vi "get_edge_attribute.vi"(7 "attribute-name":string, 8 "error in (no error)":errorcluster, 9 "default value (empty variant)":variant, 10 "edge":refnum<class "Edge.lvclass">, 11 "graph":refnum<class "Graph.lvclass">) -> (0 "error out":errorcluster, 1 "attribute-value":variant, 2 "attribute-found":bool, 3 "graph-out":refnum<class "Graph.lvclass">)   [LabVIEW 2020, in "graph.lvlib" / "Graph.lvclass"]
uses:
  Graph.lvclass
  Edge/Edge.lvclass
  Graph.lvclass/Graph.ctl
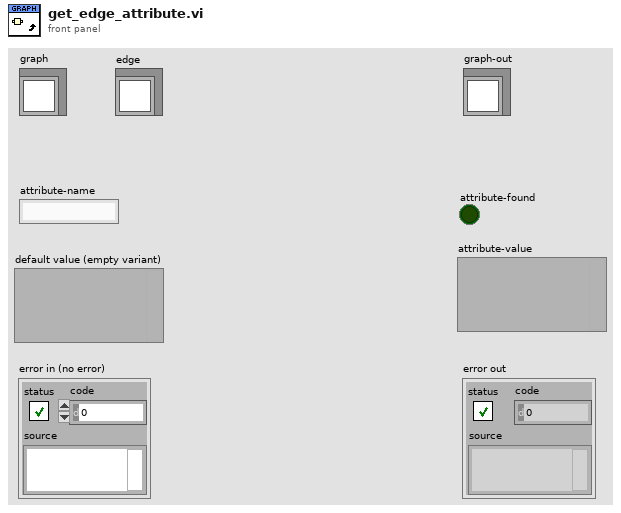
[diagram p1: front panel]
types:
  T1 = typedef "graph.lvlib/Graph.lvclass/edge-definition-cluster.ctl" = cluster{"source-id":refnum<class "ID.lvclass">, "sink-id":refnum<class "ID.lvclass">}
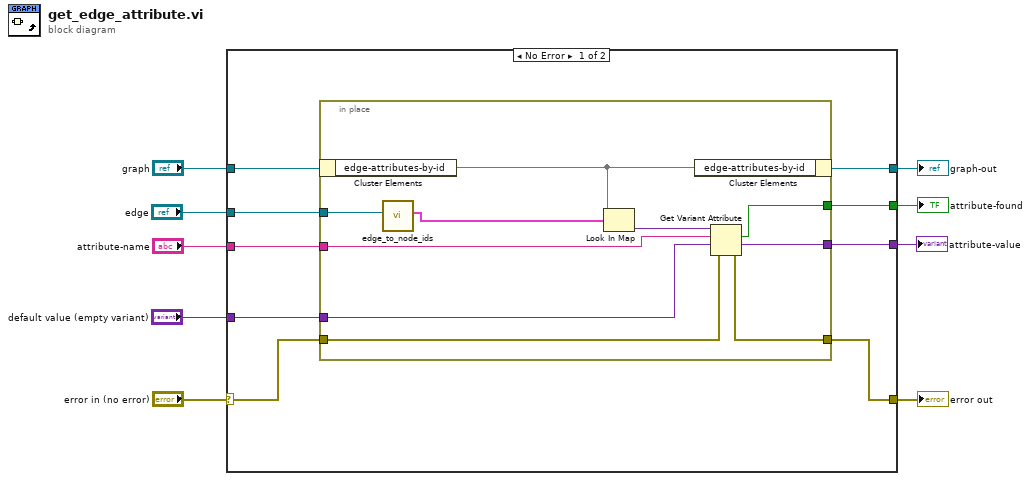
[diagram p0: block diagram]
diagram:
  n1 = case shown="No Error" "error in (no error)" {
    selector: "error in (no error)" -> [w11 w30]
    tunnel: [w10 w30] -> w8
    tunnel: [w17 w29] -> w6
    tunnel: "graph" -> [w16 w29]
    tunnel: "attribute-name" -> [w18 _]
    tunnel: "edge" -> [w15 _]
    tunnel: [w14 _] -> w3
    tunnel: "default value (empty variant)" -> [w13 _]
    tunnel: [w12 _] -> w1
    frame No Error {
      n2 = in-place {
        in-place-border: w18 -> [w26]
        in-place-border: w15 -> [w22]
        in-place-border: [w25] -> w14
        in-place-border: w13 -> [w24]
        in-place-border: [w23] -> w12
        in-place-border: w11 -> [w20]
        in-place-border: [w19] -> w10
        n3 = in-place-cluster #1(w16) -> ("edge-attributes-by-id"=w28:map{T1, variant})
        n4 = call "edge_to_node_ids.vi"("edge"=w22) -> ("node-ids-cluster"=w21:T1)  [unwired: 10 in]
        n5 = Look In Map(map=w28, key=w21) -> (value=w27:variant)  [unwired: 1 in, 1 out]
        n6 = in-place-cluster #1("edge-attributes-by-id"=w28) -> (w17:refnum<class "Graph.lvclass">)
        n7 = Get Variant Attribute(Variant=w27, name=w26, default value (empty Variant)=w24, error in=w20) -> (found=w23:bool, value=w25:variant, error out=w19:errorcluster)  [unwired: 1 out]
      }
    }
    frame Error {
    }
  }
  "error out" <- w8
  "graph-out" <- w6
  "attribute-value" <- w3
  "attribute-found" <- w1
